vi "Test Project Store INI Round Trip.vi"(8 "error in (no error)":errorcluster, 10 "Work Folder":path, 11 "Test Data Folder":path) -> (0 "error out":errorcluster, 2 "Report":string, 3 "Passed":bool)   [LabVIEW 2024]
doc: "Reads the README sample Projects.ini and Tasks.ini with Project Store-INI and writes them to a second folder: both written files must equal the samples (carriage returns ignored).\n\nInputs: Test Data Folder holds the source copies (Samples, v1); each run works in a new case folder under Work Folder. Passed is TRUE when every check passed and no error occurred; Report lists every check.\n\nGenerated by: Claude"
uses:
  Storage/Project Store-INI/Project Store-INI.lvclass
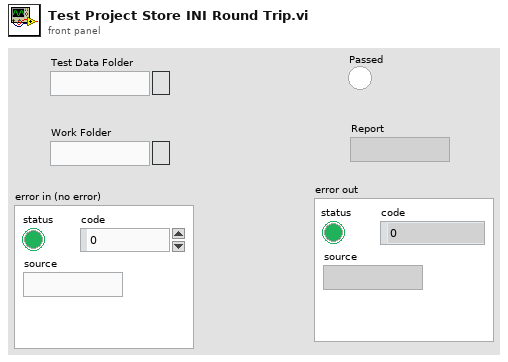
[diagram p1: front panel]
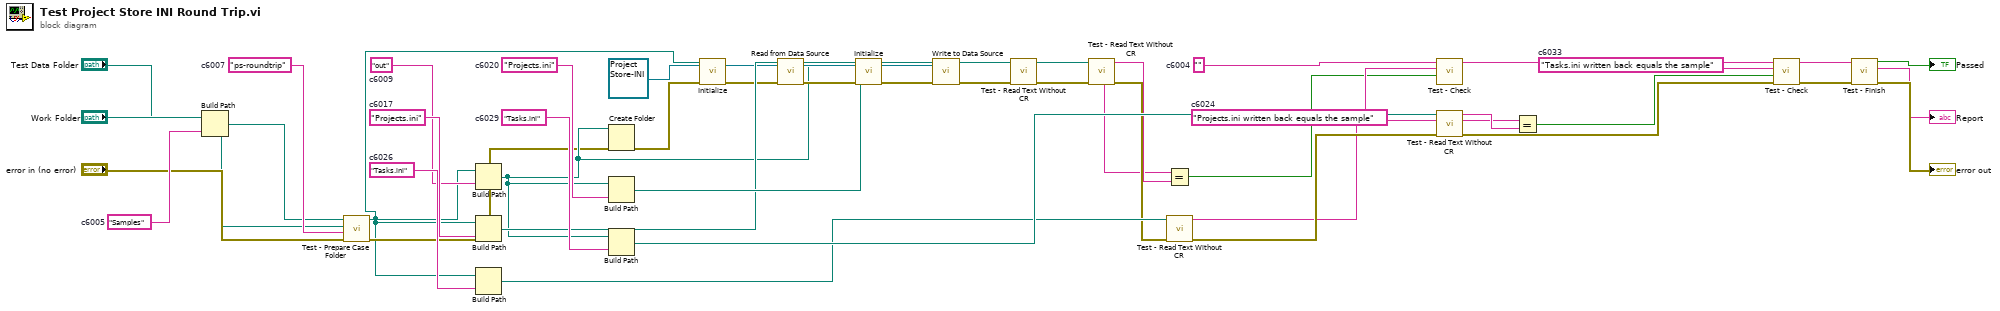
[diagram p0: block diagram]
diagram:
  w41 = "Tasks.ini written back equals the sample"  # c6033
  w36 = "Tasks.ini"  # c6029
  w32 = "Tasks.ini"  # c6026
  w30 = "Projects.ini written back equals the sample"  # c6024
  w25 = "Projects.ini"  # c6020
  w21 = "Projects.ini"  # c6017
  w10 = "out"  # c6009
  w7 = "ps-roundtrip"  # c6007
  w5 = "Samples"  # c6005
  w4 = ""  # c6004
  n1 = Build Path(base path="Test Data Folder", name or relative path=w5) -> (appended path=w6:path)
  n2 = call "Test - Prepare Case Folder.vi"("error in (no error)"="error in (no error)", "Case Name"=w7, "Work Folder"="Work Folder", "Source Folder"=w6) -> ("error out"=w9:errorcluster, "Case Folder"=w8:path)  [unwired: 6 in]
  n3 = Build Path(base path=w8, name or relative path=w10) -> (appended path=w11:path)
  n4 = Build Path(base path=w8, name or relative path=w21) -> (appended path=w22:path)
  n5 = Build Path(base path=w8, name or relative path=w32) -> (appended path=w33:path)
  n6 = Create Folder(path (use dialog)=w11, error in=w9) -> (error out=w12:errorcluster)  [unwired: 1 in, 2 out]
  n7 = Build Path(base path=w11, name or relative path=w25) -> (appended path=w26:path)
  n8 = Build Path(base path=w11, name or relative path=w36) -> (appended path=w37:path)
  n9 = call-dynamic "Initialize.vi"("Project Store in"=refnum<class "Project Store-INI.lvclass"> refnum ("Project Store-INI"), "error in (no error)"=w12, "Data Folder"=w8) -> ("error out"=w15:errorcluster, "Project Store out"=w14:refnum<class "Project Store-INI.lvclass">)  [unwired: 7 in]
  n10 = call-dynamic "Read from Data Source.vi"("Project Store in"=w14, "error in (no error)"=w15) -> ("error out"=w17:errorcluster, "Project Store out"=w16:refnum<class "Project Store-INI.lvclass">)  [unwired: 8 in]
  n11 = call-dynamic "Initialize.vi"("Project Store in"=w16, "error in (no error)"=w17, "Data Folder"=w11) -> ("error out"=w19:errorcluster, "Project Store out"=w18:refnum<class "Project Store-INI.lvclass">)  [unwired: 7 in]
  n12 = call-dynamic "Write to Data Source.vi"("Project Store in"=w18, "error in (no error)"=w19) -> ("error out"=w20:errorcluster)  [unwired: 8 in, 1 out]
  n13 = call "Test - Read Text Without CR.vi"("error in (no error)"=w20, "File"=w22) -> ("error out"=w24:errorcluster, "Text"=w23:string)  [unwired: 8 in]
  n14 = call "Test - Read Text Without CR.vi"("error in (no error)"=w24, "File"=w26) -> ("error out"=w28:errorcluster, "Text"=w27:string)  [unwired: 8 in]
  n15 = Equal?(x=w23, y=w27) -> (x = y?=w29:bool)
  n16 = call "Test - Read Text Without CR.vi"("error in (no error)"=w28, "File"=w33) -> ("error out"=w35:errorcluster, "Text"=w34:string)  [unwired: 8 in]
  n17 = call "Test - Check.vi"("Condition"=w29, "Check Name"=w30, "Report in"=w4) -> ("Report out"=w31:string)  [unwired: 7 in, 1 out]
  n18 = call "Test - Read Text Without CR.vi"("error in (no error)"=w35, "File"=w37) -> ("error out"=w39:errorcluster, "Text"=w38:string)  [unwired: 8 in]
  n19 = Equal?(x=w34, y=w38) -> (x = y?=w40:bool)
  n20 = call "Test - Check.vi"("Condition"=w40, "Check Name"=w41, "Report in"=w31) -> ("Report out"=w42:string)  [unwired: 7 in, 1 out]
  n21 = call "Test - Finish.vi"("error in (no error)"=w39, "Report"=w42) -> ("error out"=→"error out":errorcluster, "Report out"=→"Report":string, "Passed"=→"Passed":bool)  [unwired: 7 in]
